vi "GetPositionCategory.vi"(8 "error in (no error)":errorcluster, 11 "Link in":refnum<class "Link.lvclass">) -> (0 "error out":errorcluster, 2 "position":T1, 3 "Link out":refnum<class "Link.lvclass">)   [LabVIEW 2023, in "GettingStartedWindow.lvlib" / "Link.lvclass"]
uses:
  <resource>/modes/FRC/Classes/Link/Link.lvclass
  <resource>/modes/FRC/PositionCategory.ctl
  <resource>/modes/FRC/GettingStartedWindow.lvlib
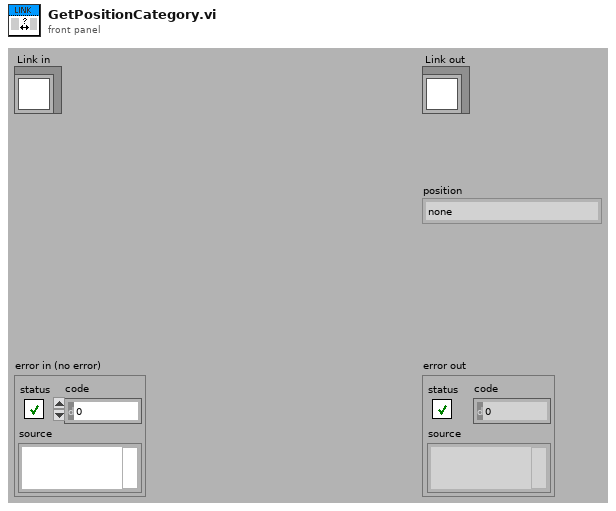
[diagram p1: front panel]
types:
  T1 = typedef "GettingStartedWindow.lvlib/PositionCategory.ctl" = enum16{"none", "column 1", "column 2", "ring"}
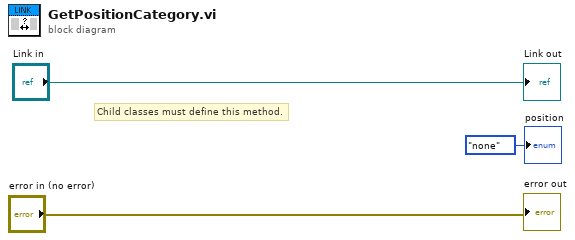
[diagram p0: block diagram]
diagram:
  # "Child classes must define this method."
  "error out" <- "error in (no error)"
  "Link out" <- "Link in"
  "position" <- PositionCategory."none" ("position")
